vi "C_Bit_Timing.vi"(6 "data sample point":dbl=80.0, 7 "nominal sample point":dbl=80.0, 8 "error in (no error)":errorcluster, 10 "data bit rate":u32=2000000, 11 "nominal bit rate":u32=500000) -> (0 "error out":errorcluster, 1 "data sample point out":dbl, 2 "nominal sample point out":dbl, 3 "Bit_Timing":T1)   [LabVIEW 2021, in "CANsub_C.lvlib"]
uses:
  CANsub_C.lvlib
  codec_vis/CANsub_Codec.lvlib
  common/Typedefs/Bit_Timing.ctl
  common/CANsub_Common.lvlib
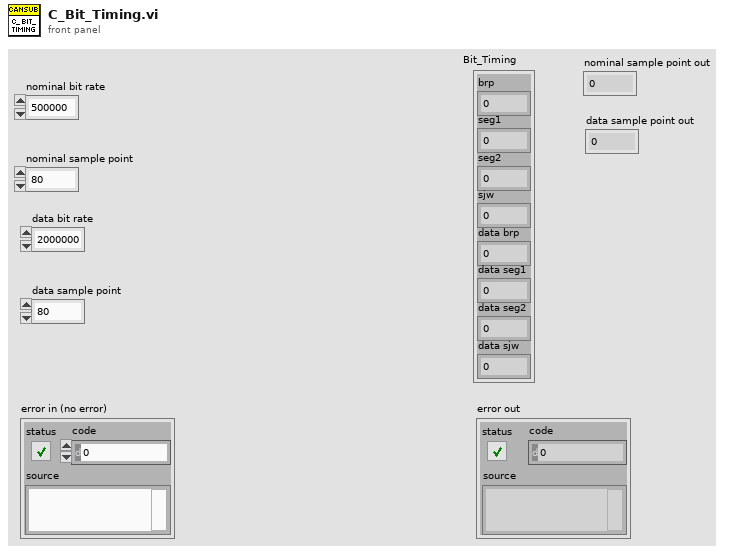
[diagram p1: front panel]
types:
  T1 = typedef "CANsub_Common.lvlib/Bit_Timing.ctl" = cluster{"brp":u16, "seg1":u16, "seg2":u16, "sjw":u16, "data brp":u16, "data seg1":u16, "data seg2":u16, "data sjw":u16}
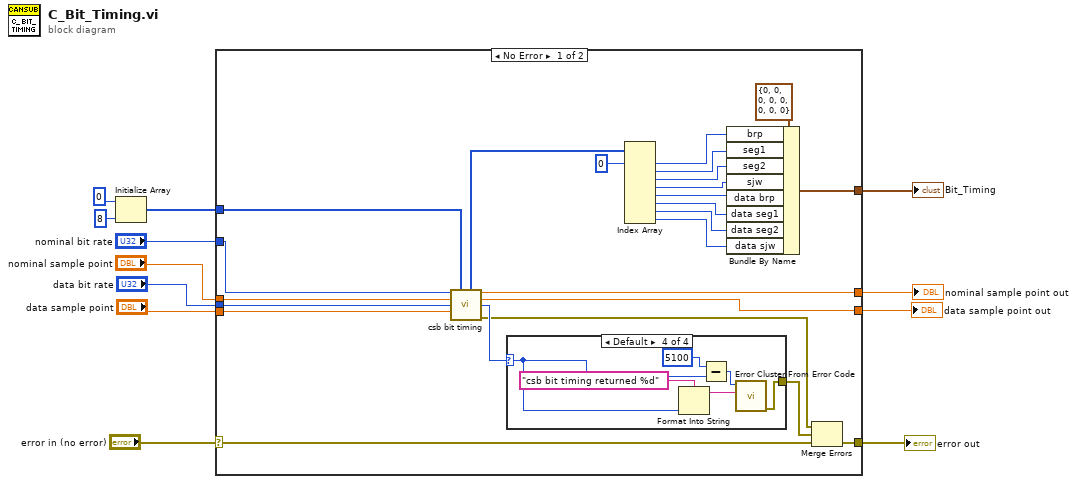
[diagram p0: block diagram]
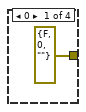
[diagram p2: hidden frame]
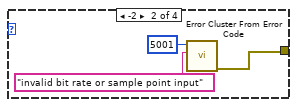
[diagram p3: hidden frame]
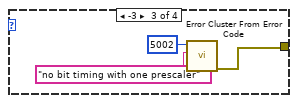
[diagram p4: hidden frame]
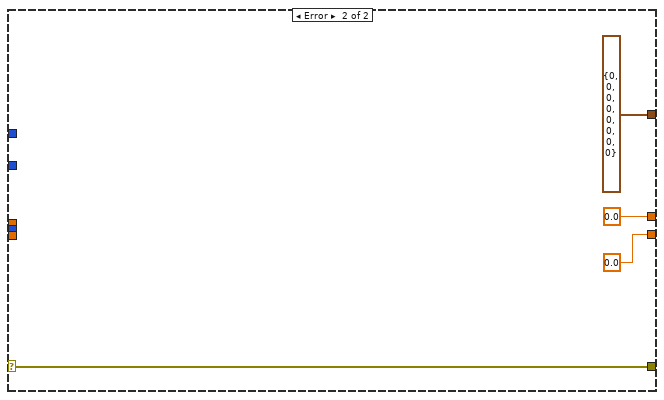
[diagram p5: hidden frame]
diagram:
  n1 = Initialize Array(u16 0, 8 ("dimension size")) -> (w10:u16[])
  n2 = case shown="No Error" "error in (no error)" {
    selector: "error in (no error)" -> [w15 w50]
    tunnel: w10 -> [w36 _]
    tunnel: "nominal bit rate" -> [w35 _]
    tunnel: "nominal sample point" -> [w34 _]
    tunnel: "data bit rate" -> [w33 _]
    tunnel: "data sample point" -> [w32 _]
    tunnel: [w31 0.0 ("nominal_sp_out")] -> w5
    tunnel: [w30 0.0 ("data_sp_out")] -> w4
    tunnel: [w19 T1 {"brp"=0, "seg1"=0, "seg2"=0, "sjw"=0, "data brp"=0, "data seg1"=0, "data seg2"=0, "data sjw"=0} ("Bit_Timing")] -> w2
    tunnel: [w18 w50] -> w1
    frame No Error {
      n3 = call "csb bit timing.vi"("nominal_bitrate"=w35, "timing"=w36, "nominal_sp"=w34, "data_bitrate"=w33, "data_sp"=w32) -> ("timing out"=w28:u16[], "nominal_sp_out"=w31:dbl, "data_sp_out"=w30:dbl, "function return"=w16:i32, "error out"=w13:errorcluster)  [unwired: 6 in]
      n4 = case shown="Default" w16 {
        selector: w16 -> [_ _ _ w46]
        tunnel: [errorcluster {"status"=FALSE, "code"=0, "source"=""} ("error constant") w38 w41 w44] -> w14
        frame 0 {
        }
        frame -2 {
          n5 = call <vilib>:"Error Cluster From Error Code.vi"("error message (\"\")"="invalid bit rate or sample point input" ("error message (\"\")"), "error code (0)"=5001) -> ("error out"=w38:errorcluster)  [unwired: 7 in]
        }
        frame -3 {
          n6 = call <vilib>:"Error Cluster From Error Code.vi"("error message (\"\")"="no bit timing with one prescaler" ("error message (\"\")"), "error code (0)"=5002) -> ("error out"=w41:errorcluster)  [unwired: 7 in]
        }
        frame Default {
          n7 = Format Into String(format string="csb bit timing returned %d", w46) -> (resulting string=w48:string)  [unwired: 2 in, 1 out]
          n8 = Subtract(x=5100, y=w46) -> (x-y=w45:i32)
          n9 = call <vilib>:"Error Cluster From Error Code.vi"("error message (\"\")"=w48, "error code (0)"=w45) -> ("error out"=w44:errorcluster)  [unwired: 7 in]
        }
      }
      n10 = Index Array(array=w28, index #1=0 ("index")) -> (element #1=w27:u16, element #2=w26:u16, element #3=w25:u16, element #4=w24:u16, element #5=w23:u16, element #6=w22:u16, element #7=w21:u16, element #8=w20:u16)  [unwired: 7 in]
      n11 = Bundle By Name(cluster=T1 {"brp"=0, "seg1"=0, "seg2"=0, "sjw"=0, "data brp"=0, "data seg1"=0, "data seg2"=0, "data sjw"=0} ("Bit_Timing"), "brp"=w27, "seg1"=w26, "seg2"=w25, "sjw"=w24, "data brp"=w23, "data seg1"=w22, "data seg2"=w21, "data sjw"=w20) -> (w19:T1)
      n12 = Merge Errors(w13, w14, w15) -> (w18:errorcluster)
    }
    frame Error {
    }
  }
  "Bit_Timing" <- w2
  "nominal sample point out" <- w5
  "data sample point out" <- w4
  "error out" <- w1
